vi "CSE ISP - post-execution operations.vi"(7 "loaded functions":string[](array[string]), 8 "error in":errorcluster, 9 "ISP menu":refnum<k9>, 10 "Callback VI RefNum":T1, 11 "CSE RefNum":T2) -> (0 "error out":errorcluster, 3 "dup CSE RefNum":T2)   [LabVIEW 2021]
doc: "::: CalcExpress Toolkit :::\nCopyright (c) 2000-2026 Konstantin Shifershteyn. All rights reserved."
uses:
  vi.lib/addons/CalcExpress/cse.llb/CSE Instance RefNum.ctl
  vi.lib/addons/CalcExpress/cse.llb/CSE Callback VI RefNum.ctl
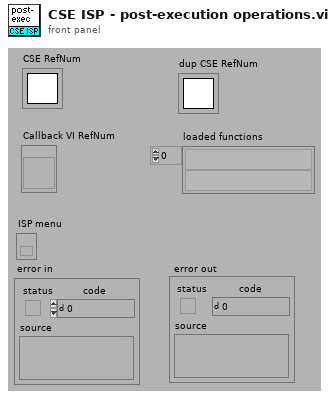
[diagram p1: front panel]
types:
  T1 = typedef "CSE Callback VI RefNum.ctl" = refnum<vi>
  T2 = typedef "CSE Instance RefNum.ctl" = refnum<k1>
  T3 = cluster{"reuse context":bool, "reuse variables":bool, "keep variables":bool}
  T4 = cluster{"unload FuncVIs":bool, "debug: line mode":bool}
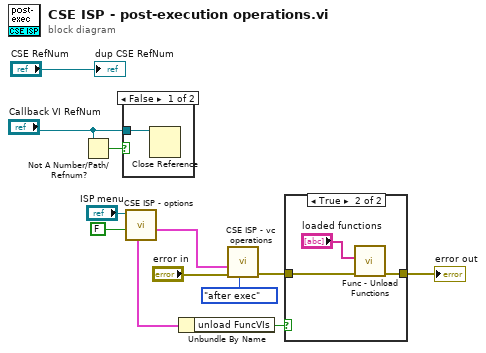
[diagram p0: block diagram]
diagram:
  n1 = Not A Number/Path/Refnum?(number/path/refnum="Callback VI RefNum") -> (NaN/Path/Refnum?=w3:bool)
  n2 = case shown="False" w3 {
    tunnel: "Callback VI RefNum" -> [w13 _]
    frame False {
      n3 = Close Reference(reference=w13) -> ()  [unwired: 1 in, 1 out]
    }
    frame True {
    }
  }
  n4 = call "CSE ISP - options.vi"("enable menu (T)"=FALSE, "ISP menu"="ISP menu") -> ("VM params"=w10:T3, "misc params"=w9:T4)  [unwired: 2 in, 6 out]
  n5 = Unbundle By Name(w9) -> ("unload FuncVIs"=w1:bool)
  n6 = call "CSE ISP - vc operations.vi"("cmd"=enum16{"before exec", "after exec", "init"}."after exec", "error in"="error in", "params"=w10) -> ("error out"=w8:errorcluster)  [unwired: 7 in, 1 out]
  n7 = case shown="True" w1 {
    tunnel: w8 -> [w14 w16]
    tunnel: [w14 w15] -> w7
    frame False {
    }
    frame True {
      n8 = call "Func - Unload Functions.vi"("error in"=w16, "Array of func names"="loaded functions") -> ("error out"=w15:errorcluster)  [unwired: 7 in]
    }
  }
  "error out" <- w7
  "dup CSE RefNum" <- "CSE RefNum"
